vi "Set Waveform formats.vi"(8 "error in (no error)":errorcluster, 9 "Theta":refnum<vi>, 10 "R":refnum<vi>, 11 "State In":T1 caption="State") -> (0 "error out":errorcluster, 3 "State Out":T1 caption="State")   [LabVIEW 2012, in "Vector Function Generator.xctl"]
doc: "Pass through waveform methods to set format and displays, paying attention to polar or cartesian modes"
uses:
  Vector Function Generator.xctl
  Vector State.ctl
  <userlib>/_LAVAcr/User_Interface/XControls/Waveform_XControl/Waveform Control.xctl
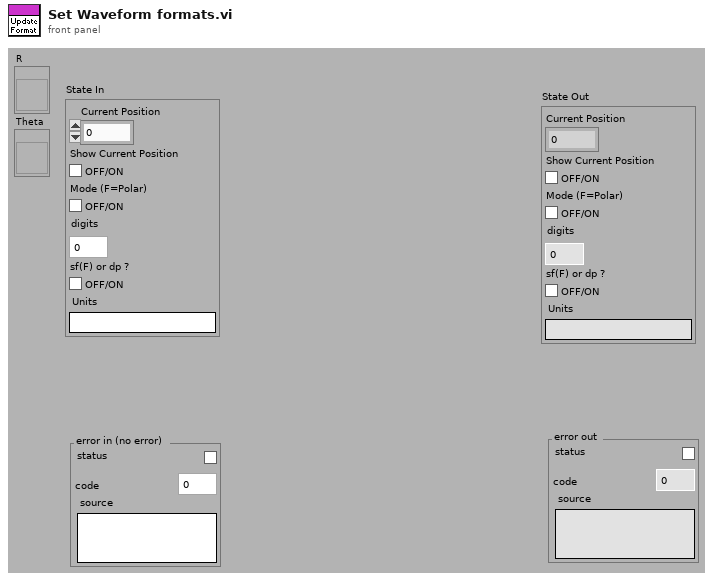
[diagram p1: front panel]
types:
  T1 = typedef "Vector Function Generator.xctl/Vector State.ctl" = cluster{"Current Position":i32, "Show Current Position":bool, "Mode (F=Polar)":bool, "digits":i32, "sf(F) or dp ?":bool, "Units":string}
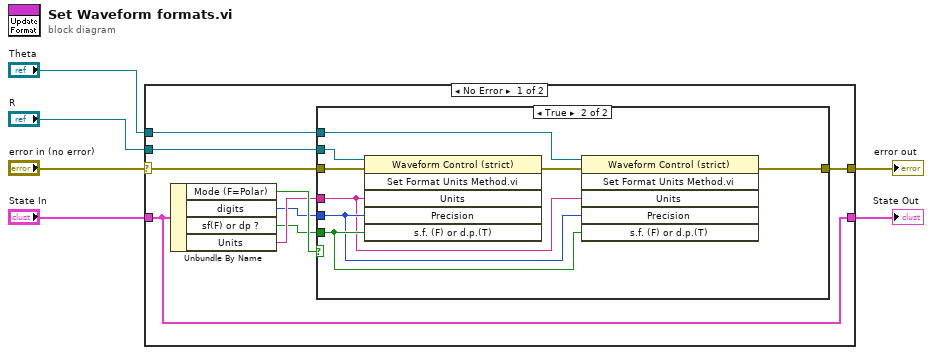
[diagram p0: block diagram]
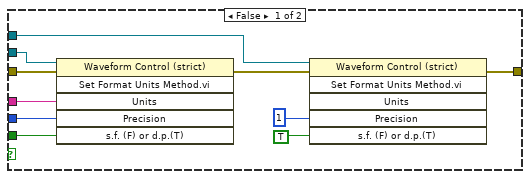
[diagram p2: hidden frame]
diagram:
  n1 = case shown="No Error" "error in (no error)" {
    selector: "error in (no error)" -> [w9 w34]
    tunnel: "State In" -> [w7 w35]
    tunnel: "R" -> [w14 _]
    tunnel: "Theta" -> [w10 _]
    tunnel: [w8 w34] -> w2
    tunnel: [w7 w35] -> w1
    frame No Error {
      n2 = Unbundle By Name(w7) -> ("Mode (F=Polar)"=w15:bool, "digits"=w12:i32, "sf(F) or dp ?"=w11:bool, "Units"=w13:string)
      n3 = case shown="True" w15 {
        tunnel: w14 -> [w25 w33]
        tunnel: w13 -> [w24 w26]
        tunnel: w12 -> [w23 w27]
        tunnel: w11 -> [w22 w28]
        tunnel: w10 -> [w18 w31]
        tunnel: w9 -> [w17 w30]
        tunnel: [w16 w29] -> w8
        frame False {
          n4 = invoke class="Waveform Control (strict)" method="Set Format Units Method.vi"(reference=w25, error in=w17, "Units"=w24, "Precision"=w23, "s.f. (F) or d.p.(T)"=w22) -> (error out=w21:errorcluster)  [unwired: 1 in, 5 out]
          n5 = invoke class="Waveform Control (strict)" method="Set Format Units Method.vi"(reference=w18, error in=w21, "Precision"=1, "s.f. (F) or d.p.(T)"=TRUE) -> (error out=w16:errorcluster)  [unwired: 2 in, 5 out]
        }
        frame True {
          n6 = invoke class="Waveform Control (strict)" method="Set Format Units Method.vi"(reference=w33, error in=w30, "Units"=w26, "Precision"=w27, "s.f. (F) or d.p.(T)"=w28) -> (error out=w32:errorcluster)  [unwired: 1 in, 5 out]
          n7 = invoke class="Waveform Control (strict)" method="Set Format Units Method.vi"(reference=w31, error in=w32, "Units"=w26, "Precision"=w27, "s.f. (F) or d.p.(T)"=w28) -> (error out=w29:errorcluster)  [unwired: 1 in, 5 out]
        }
      }
    }
    frame Error {
    }
  }
  "error out" <- w2
  "State Out" <- w1
